vi "Button was Pressed.vi"(8 "error in":errorcluster, 10 "Button Pressed":enum16{"Yes", "No", "Maybe"}(ring)) -> (0 "error out":errorcluster)   [LabVIEW 2024, in "Mysterious DQMH Module.lvlib"]
doc: "This event broadcasts which button was pressed\n\n_____\nCreated using DQMH Framework: Event Scripter 7.1.2.1547."
uses:
  Mysterious DQMH Module.lvlib
  Button was Pressed Argument--cluster.ctl
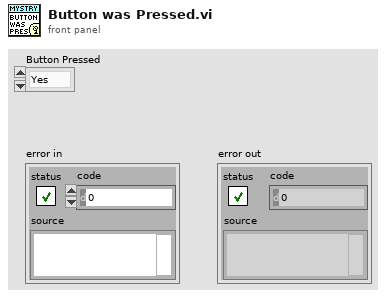
[diagram p1: front panel]
types:
  T1 = typedef "Mysterious DQMH Module.lvlib/Button was Pressed Argument--cluster.ctl" = cluster{"Button Pressed":enum16{"Yes", "No", "Maybe"}}
  T2 = typedef "Mysterious DQMH Module.lvlib/Broadcast Events--cluster.ctl" = cluster{"Module Did Init":refnum<user-event>, "Status Updated":refnum<user-event>, "Error Reported":refnum<user-event>, "Module Did Stop":refnum<user-event>, "Update Module Execution Status":refnum<user-event>, "Button was Pressed":refnum<user-event>}
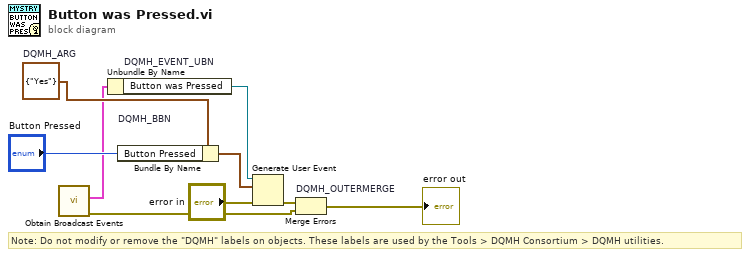
[diagram p0: block diagram]
diagram:
  w4 = T1 {"Button Pressed"=enum."Yes"}  # DQMH_ARG
  # "Note: Do not modify or remove the \"DQMH\" labels on objects. These labels are used by the Tools > DQMH Consortium > DQMH utilities."
  n1 = call "Obtain Broadcast Events.vi"() -> ("error out"=w2:errorcluster, "Mysterious DQMH Module Broadcast Events"=w1:T2)  [unwired: 10 in]
  n2 = Unbundle By Name "DQMH_EVENT_UBN"(w1) -> ("Button was Pressed"=w6:refnum<user-event>)
  n3 = Bundle By Name "DQMH_BBN"(cluster=w4, "Button Pressed"="Button Pressed") -> (w7:T1)
  n4 = Generate User Event(user event=w6, event data cluster=w7, error in="error in") -> (error out=w5:errorcluster)  [unwired: 1 in, 1 out]
  n5 = Merge Errors "DQMH_OUTERMERGE"(w5, w2) -> (→"error out":errorcluster)
